vi "VM - List of Aliases.vi"(8 "error in":errorcluster, 9 "reverse? (F)":bool, 10 "sort":T1(ring)) -> (0 "error out":errorcluster, 3 "aliases info":T2[](array[typedef]))   [LabVIEW 2021]
doc: "This VI returns information about all active aliases and associated variables. Refer to the VI help for more details.\n\n::: CalcExpress Toolkit :::\nCopyright (c) 2000-2026 Konstantin Shifershteyn. All rights reserved."
uses:
  cetypes.llb/VarMan Alias Info Cluster.ctl
  cetypes.llb/VarMan Variable Context Handle.ctl
  cetypes.llb/VarMan Error Code.ctl
  cersrc/celveng32.dll
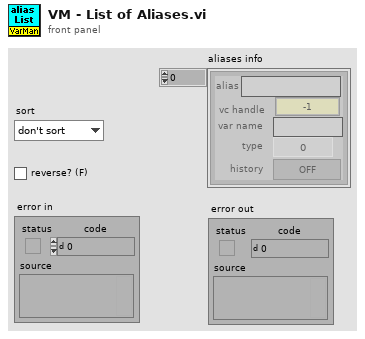
[diagram p1: front panel]
types:
  T1 = enum16{"don't sort", "alias", "vc handle", "name", "type"}
  T2 = typedef "VarMan Alias Info Cluster.ctl" = cluster{"alias":string, "vc handle":T3, "var name":string, "type":u32, "history":bool}
  T3 = typedef "VarMan Variable Context Handle.ctl" = i32
  T4 = typedef "VarMan Error Code.ctl" = u16
  T5 = cluster{"alias":string, "vc handle":T3, "name":string, "type":u32, "has history":bool}[]
  T6 = cluster{"alias":string, "vc handle":T3, "name":string, "type":u32, "has history":bool}
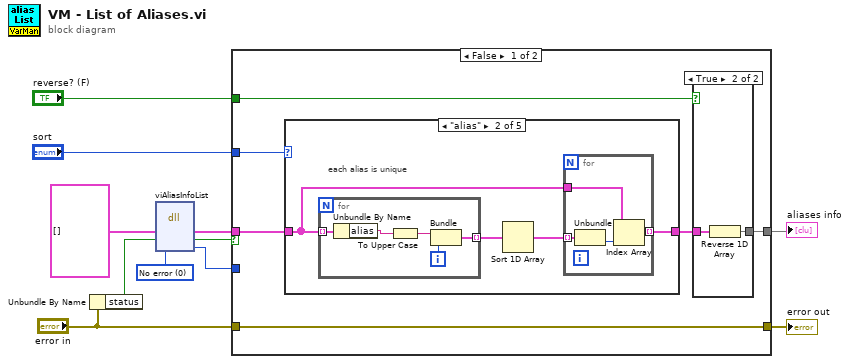
[diagram p0: block diagram]
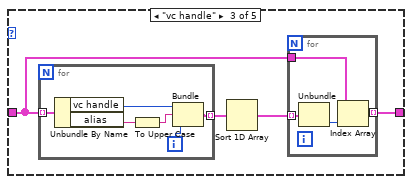
[diagram p4: hidden frame]
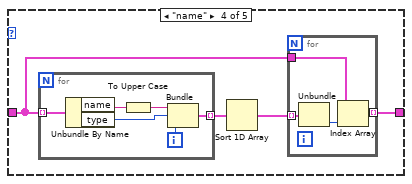
[diagram p5: hidden frame]
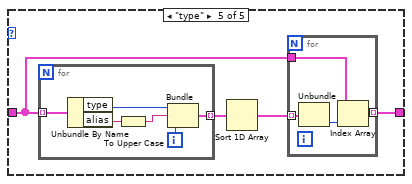
[diagram p6: hidden frame]
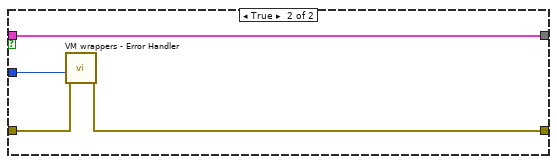
[diagram p7: hidden frame]
diagram:
  w3 = T4 0 items=["No error", "Invalid variable type", "Variable not found", "Variable already exists", "Invalid context handle", "Input error", "Invalid data format", "No history attached", "History already attached", "Invalid history parameters", "Wrong variable name", "Wrong alias name", "Non-unique alias", "Alias not found", "No alias associated", "Alias already associated", "Wrong context name", "Non-unique context name", "Context name not found", "Invalid parameter", "Generic error", "Memory Full", "Unrecognized LV error", "Unknown error code"] ("VarMan error")
  n1 = Unbundle By Name("error in") -> ("status"=w6:bool)
  n2 = dll-call lib="C:/LV Projects/CalcExpress 40 LV2021/vi.lib/addons/CalcExpress/cersrc/celveng*.dll" fn="viAliasInfoList"("aliasList"=T5 [] ("list of aliases"), "errf"=w6, "errc"=w3) -> ("aliasList"=w4:T5, "errf"=w7:bool, "errc"=w8:T4)  [unwired: 4 in, 2 out]
  n3 = case shown="False" w7 {
    tunnel: [w16 w80] -> w9
    tunnel: w4 -> [w15 w80]
    tunnel: w8 -> [_ w77]
    tunnel: [w14 w78] -> w10
    tunnel: "error in" -> [w14 w79]
    tunnel: "sort" -> [w13 _]
    tunnel: "reverse? (F)" -> [w12 _]
    frame False {
      n4 = case shown="\"alias\"" w13 {
        tunnel: [w21 w25 w38 w52 w66] -> w17
        tunnel: w15 -> [w21 w22 w35 w49 w63]
        frame "don't sort" {
        }
        frame "alias" {
          # "each alias is unique"
          n5 = for {
            tunnel: w22 -> [w34] mode=indexing
            tunnel: [w30] -> w23 mode=indexing
            i -> [w31]
            n6 = Unbundle By Name(w34) -> ("alias"=w33:string)
            n7 = To Upper Case(1:w33) -> (0:w32:string)
            n8 = Bundle(w32, w31) -> (w30:cluster{string, i32})  [unwired: 1 in]
          }
          n9 = Sort 1D Array(array=w23) -> (sorted array=w24:cluster{string, i32}[])
          n10 = for {
            tunnel: w24 -> [w29] mode=indexing
            tunnel: [w28] -> w25 mode=indexing
            tunnel: w22 -> [w26]
            n11 = Unbundle(w29) -> (w27:i32)  [unwired: 1 out]
            n12 = Index Array(array=w26, index=w27) -> (element=w28:T6)
          }
        }
        frame "vc handle" {
          n13 = for {
            tunnel: w35 -> [w48] mode=indexing
            tunnel: [w44] -> w36 mode=indexing
            i -> [w45]
            n14 = Unbundle By Name(w48) -> ("vc handle"=w43:T3, "alias"=w47:string)
            n15 = To Upper Case(1:w47) -> (0:w46:string)
            n16 = Bundle("vc handle"=w43, w46, w45) -> (w44:cluster{"vc handle":T3, string, i32})  [unwired: 1 in]
          }
          n17 = Sort 1D Array(array=w36) -> (sorted array=w37:cluster{"vc handle":T3, string, i32}[])
          n18 = for {
            tunnel: w37 -> [w42] mode=indexing
            tunnel: [w41] -> w38 mode=indexing
            tunnel: w35 -> [w39]
            n19 = Unbundle(w42) -> (w40:i32)  [unwired: 2 out]
            n20 = Index Array(array=w39, index=w40) -> (element=w41:T6)
          }
        }
        frame "name" {
          n21 = for {
            tunnel: w49 -> [w62] mode=indexing
            tunnel: [w58] -> w50 mode=indexing
            i -> [w59]
            n22 = Unbundle By Name(w62) -> ("name"=w61:string, "type"=w57:u32)
            n23 = To Upper Case(1:w61) -> (0:w60:string)
            n24 = Bundle(w60, "type"=w57, w59) -> (w58:cluster{string, "type":u32, i32})  [unwired: 1 in]
          }
          n25 = Sort 1D Array(array=w50) -> (sorted array=w51:cluster{string, "type":u32, i32}[])
          n26 = for {
            tunnel: w51 -> [w56] mode=indexing
            tunnel: [w55] -> w52 mode=indexing
            tunnel: w49 -> [w53]
            n27 = Unbundle(w56) -> (w54:i32)  [unwired: 2 out]
            n28 = Index Array(array=w53, index=w54) -> (element=w55:T6)
          }
        }
        frame "type" {
          n29 = for {
            tunnel: w63 -> [w76] mode=indexing
            tunnel: [w74] -> w64 mode=indexing
            i -> [w75]
            n30 = Unbundle By Name(w76) -> ("type"=w71:u32, "alias"=w73:string)
            n31 = To Upper Case(1:w73) -> (0:w72:string)
            n32 = Bundle("type"=w71, w72, w75) -> (w74:cluster{"type":u32, string, i32})  [unwired: 1 in]
          }
          n33 = Sort 1D Array(array=w64) -> (sorted array=w65:cluster{"type":u32, string, i32}[])
          n34 = for {
            tunnel: w65 -> [w70] mode=indexing
            tunnel: [w69] -> w66 mode=indexing
            tunnel: w63 -> [w67]
            n35 = Unbundle(w70) -> (w68:i32)  [unwired: 2 out]
            n36 = Index Array(array=w67, index=w68) -> (element=w69:T6)
          }
        }
      }
      n37 = case shown="True" w12 {
        tunnel: w17 -> [w18 w20]
        tunnel: [w18 w19] -> w16
        frame False {
        }
        frame True {
          n38 = Reverse 1D Array(array=w20) -> (reversed array=w19:T5)
        }
      }
    }
    frame True {
      n39 = call "VM wrappers - Error Handler.vi"("error before"=w79, "VarMan error"=w77) -> ("error out"=w78:errorcluster)  [unwired: 8 in, 1 out]
    }
  }
  "error out" <- w10
  "aliases info" <- w9
